vi "Encode TextString.vi"(7 "Convert to UTF8? (T)":bool=TRUE, 10 "Text String":string) -> (3 "Length-Prefixed Field":u8[](array[numeric]) format="%08b")   [LabVIEW 2013, in "MQTT_Control_Packets.lvlib" / "ControlPacket.lvclass"]
uses:
  ControlPacket.lvclass
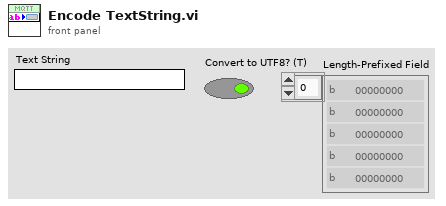
[diagram p1: front panel]
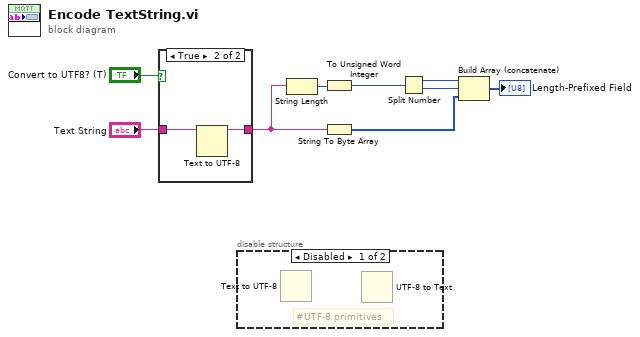
[diagram p0: block diagram]
diagram:
  n1 = case shown="True" "Convert to UTF8? (T)" {
    tunnel: [w10 w12] -> w5
    tunnel: "Text String" -> [w10 w11]
    frame False {
    }
    frame True {
      n2 = Text to UTF-8(11:w11) -> (3:w12:string)  [unwired: 1 in, 1 out]
    }
  }
  n3 = disable-structure shown="Disabled" {
    frame Disabled {
      # "#UTF-8 primitives"
      n4 = Text to UTF-8() -> ()  [unwired: 2 in, 2 out]
      n5 = UTF-8 to Text() -> ()  [unwired: 2 in, 2 out]
    }
    frame Enabled {
    }
  }
  n6 = String Length(string=w5) -> (length=w8:i32)
  n7 = To Unsigned Word Integer(number=w8) -> (unsigned 16bit integer=w2:u16)
  n8 = String To Byte Array(string=w5) -> (unsigned byte array=w4:u8[])
  n9 = Split Number(x=w2) -> (hi(x)=w7:u8, lo(x)=w6:u8)
  n10 = Build Array (concatenate)(w7, w6, w4) -> (→"Length-Prefixed Field":u8[])
